vi "CANSUB Read Xnet Frames.vi"(8 "error in (no error)":errorcluster, 10 "nBufferSize":i32=65536, 11 "nClientID":i16) -> (0 "error out":errorcluster, 1 "function return":i32, 2 "pFrameCount":i32, 3 "pBuffer":u8[](array[numeric]))   [LabVIEW 2020, in "cansub_rp1210.lvlib"]
doc: "long __stdcall CANSUB_ReadXnetFrames(short nClientID, unsigned char pBuffer[], long nBufferSize, long *pFrameCount);"
uses:
  cansub_rp1210.lvlib
  cansub_lv64.dll
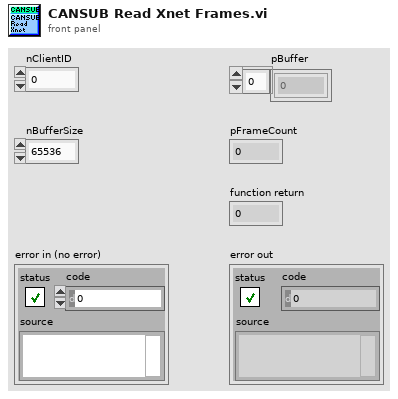
[diagram p1: front panel]
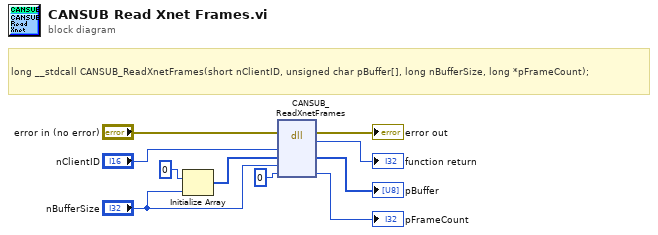
[diagram p0: block diagram]
diagram:
  # "long __stdcall CANSUB_ReadXnetFrames(short nClientID, unsigned char pBuffer[], long nBufferSize, long *pFrameCount);"
  n1 = Initialize Array(u8 0 ("element"), "nBufferSize") -> (w8:u8[])
  n2 = dll-call lib="C:/cansub-lv/library/cansub_lv*.*" fn="CANSUB_ReadXnetFrames"(error in="error in (no error)", "nClientID"="nClientID", "pBuffer"=w8, "nBufferSize"="nBufferSize", "pFrameCount"=0) -> (error out=→"error out":errorcluster, "return type"=→"function return":i32, "pBuffer"=→"pBuffer":u8[], "pFrameCount"=→"pFrameCount":i32)  [unwired: 4 in, 1 out]
